vi "Display Probe Final.vi"(0 "x":dbl) -> (4 "negative?":bool, 6 "joined":string, 8 "array":dbl[](array[numeric]))   [LabVIEW 2026]
doc: "Probe: constant labels, whitespace string, array constant, error constant, loop stop terminal, comparison with zero."
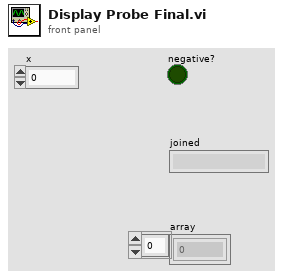
[diagram p1: front panel]
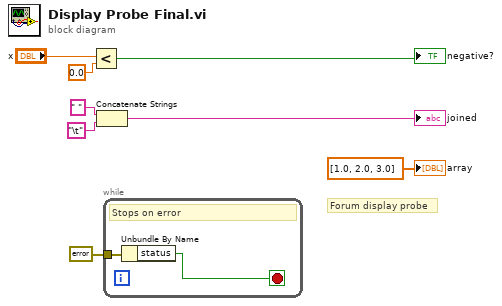
[diagram p0: block diagram]
diagram:
  # "Forum display probe"
  n1 = Less?(x="x", y=0.0 ("Zero")) -> (x < y?=→"negative?":bool)
  n2 = Concatenate Strings(" " ("separator"), "\t" ("tab")) -> (→"joined":string)
  n3 = while {
    tunnel: errorcluster {"status"=FALSE, "code"=0, "source"=""} ("no error") -> [w9]
    stop <- w10 stop-if-true
    # "Stops on error"
    n4 = Unbundle By Name(w9) -> ("status"=w10:bool)
  }
  "array" <- dbl[] [1.0, 2.0, 3.0] ("values")
